vi "gu_open_file_dialog.vi"(7 "Prompt":T1, 8 "error in":errorcluster, 10 "Multi-select":bool, 11 "Start Path":T1) -> (0 "error out":errorcluster, 1 "Cancelled":bool, 2 "Encoded Paths":T1[](array[typedef]), 3 "Encoded Path":T1)   [LabVIEW 2020, in "G-Unicode.lvlib"]
uses:
  G-Unicode.lvlib
  Types/Encoded UTF-8 String.ctl
  Memory/Copy String.vi/4d47babd-4a2d-4eb7-b91b-7e707d692665.vi
  gu_free.vi
  <vilib>/Utility/error.llb/Error Cluster From Error Code.vi
  lib/g_unicode_32.dll
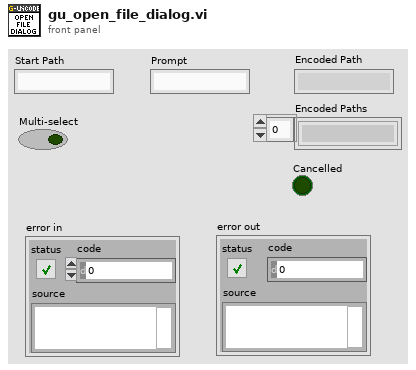
[diagram p1: front panel]
types:
  T1 = typedef "G-Unicode.lvlib/Encoded UTF-8 String.ctl" = string
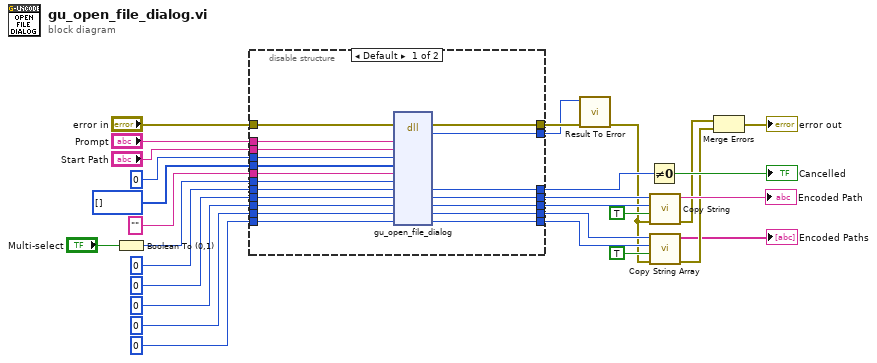
[diagram p0: block diagram]
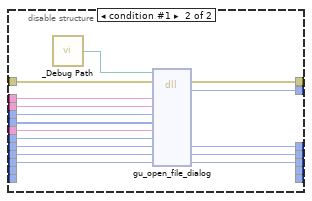
[diagram p2: hidden frame]
diagram:
  n1 = Boolean To (0,1)(Boolean="Multi-select") -> (0, 1=w2:i16)
  n2 = disable-structure shown="Default" {
    disable-tunnel: "error in" -> [w48 w64]
    disable-tunnel: [w47 w63] -> w14
    disable-tunnel: "Prompt" -> [w46 w62]
    disable-tunnel: "Start Path" -> [w45 w61]
    disable-tunnel: 0 ("num_filter_patterns") -> [w44 w60]
    disable-tunnel: i64[] [] ("filter_patterns") -> [w43 w59]
    disable-tunnel: "" ("filter_description") -> [w42 w58]
    disable-tunnel: w2 -> [w41 w57]
    disable-tunnel: i64 0 ("path_pointer") -> [w40 w56]
    disable-tunnel: 0 ("path_length") -> [w39 w55]
    disable-tunnel: [w38 w54] -> w25
    disable-tunnel: [w37 w53] -> w24
    disable-tunnel: [w35 w50] -> w23
    disable-tunnel: 0 ("path_pointer") -> [w36 w49]
    disable-tunnel: [w34 w51] -> w13
    disable-tunnel: i64 0 ("path_pointer") -> [w33 _]
    disable-tunnel: 0 ("path_length") -> [w32 _]
    disable-tunnel: [w31 _] -> w9
    disable-tunnel: [w30 _] -> w8
    frame condition #0 (active) {
      n3 = dll-call lib="C:/github/dataflowg/g-unicode/src/LabVIEW/G-Unicode/lib/g_unicode_*.*" fn="gu_open_file_dialog"(error in=w48, "title"=w46, "default_path"=w45, "num_filter_patterns"=w44, "filter_patterns"=w43, "filter_description"=w42, "allow_multi_select"=w41, "cancelled"=w36, "path_pointer"=w40, "path_length"=w39, "paths_pointer"=w33, "num_paths"=w32) -> (error out=w47:errorcluster, "result"=w34:i32, "cancelled"=w35:i32, "path_pointer"=w38:i64, "path_length"=w37:i32, "paths_pointer"=w31:i64, "num_paths"=w30:i32)  [unwired: 8 in, 1 out]
    }
    frame condition #1 {
      n4 = call "_Debug Path.vi"() -> ("Debug Path"=w52:path)
      n5 = dll-call lib="?" fn="gu_open_file_dialog"(path in=w52, error in=w64, "title"=w62, "default_path"=w61, "num_filter_patterns"=w60, "filter_patterns"=w59, "filter_description"=w58, "allow_multi_select"=w57, "cancelled"=w49, "path_pointer"=w56, "path_length"=w55) -> (error out=w63:errorcluster, "result"=w51:i32, "cancelled"=w50:i32, "path_pointer"=w54:i64, "path_length"=w53:i32)  [unwired: 7 in, 1 out]
    }
  }
  n6 = call "Result To Error.vi"("error in (no error)"=w14, "Result Code"=w13) -> ("error out"=w7:errorcluster)  [unwired: 9 in]
  n7 = Not Equal To 0?(x=w23) -> (x != 0?=→"Cancelled":bool)
  n8 = call "Copy String.vi"("error in"=w7, "free (F)"=TRUE, "size"=w24, "pointer"=w25) -> ("error out"=w6:errorcluster, "string"=→"Encoded Path":string)  [unwired: 6 in]
  n9 = call "Copy String Array.vi"("error in"=w7, "free (F)"=TRUE, "size"=w8, "pointer"=w9) -> ("error out"=w5:errorcluster, "Strings"=→"Encoded Paths":string[])  [unwired: 6 in]
  n10 = Merge Errors(w6, w5) -> (→"error out":errorcluster)
